vi "Read_tcx_file.vi"(8 "error in (no error)":errorcluster, 11 "file path":path) -> (0 "error out":errorcluster, 2 "Bpm":i32[](array[numeric]), 3 "Time":timestamp[](array[timestamp]))   [LabVIEW 2025]
uses:
  <vilib>/regexp/Match Regular Expression.xnode
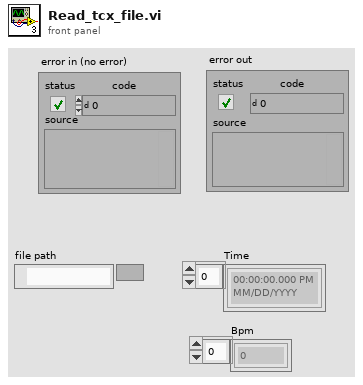
[diagram p1: front panel]
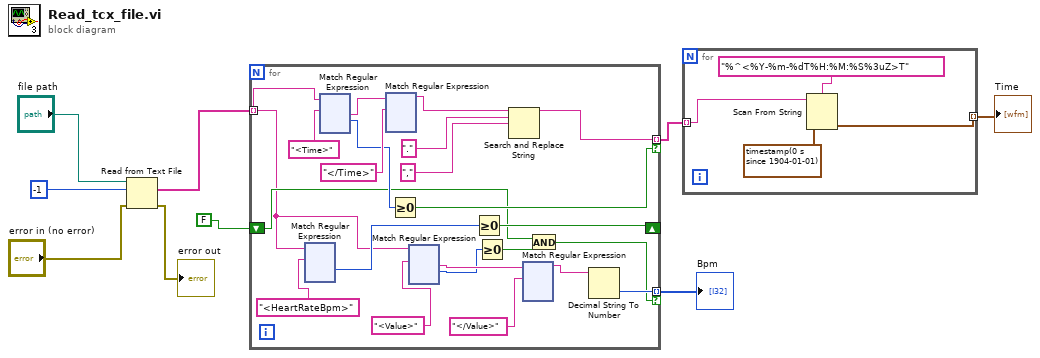
[diagram p0: block diagram]
diagram:
  n1 = Read from Text File(file (use dialog)="file path", count=-1, error in="error in (no error)") -> (text=w7:string[], error out=→"error out":errorcluster)  [unwired: 1 in, 2 out]
  n2 = for {
    tunnel: w7 -> [w10] mode=indexing
    tunnel: [w12] -> w2 mode=indexing if=w24
    shift-right: [w19] -> _
    shift-left: FALSE -> [w16]
    tunnel: [w14] -> w3 mode=indexing if=w13
    n3 = xnode "Match Regular Expression"("input string"=w10, "regular expression"="<HeartRateBpm>") -> ("offset past match"=w11:i32)  [unwired: 4 in, 4 out]
    n4 = xnode "Match Regular Expression"("input string"=w10, "regular expression"="<Time>") -> ("after match"=w30:string, "offset past match"=w25:i32)  [unwired: 4 in, 3 out]
    n5 = xnode "Match Regular Expression"("input string"=w30, "regular expression"="</Time>") -> ("before match"=w28:string)  [unwired: 4 in, 4 out]
    n6 = Greater Or Equal To 0?(x=w25) -> (x >= 0?=w24:bool)
    n7 = xnode "Match Regular Expression"("input string"=w10, "regular expression"="<Value>") -> ("after match"=w21:string, "offset past match"=w17:i32)  [unwired: 4 in, 3 out]
    n8 = Greater Or Equal To 0?(x=w11) -> (x >= 0?=w19:bool)
    n9 = Greater Or Equal To 0?(x=w17) -> (x >= 0?=w15:bool)
    n10 = Search and Replace String(input string=w28, search string=".", replace string=",") -> (result string=w12:string)  [unwired: 5 in, 3 out]
    n11 = xnode "Match Regular Expression"("input string"=w21, "regular expression"="</Value>") -> ("before match"=w18:string)  [unwired: 4 in, 4 out]
    n12 = And(x=w16, y=w15) -> (x .and. y?=w13:bool)
    n13 = Decimal String To Number(string=w18) -> (number=w14:i32)  [unwired: 2 in, 1 out]
  }
  "Bpm" <- w3
  n14 = for {
    tunnel: w2 -> [w619] mode=indexing
    tunnel: [w618] -> w1 mode=indexing
    n15 = Scan From String(format string="%^<%Y-%m-%dT%H:%M:%S%3uZ>T", input string=w619, default 1=timestamp(0 s since 1904-01-01)) -> (output 1=w618:timestamp)  [unwired: 2 in, 3 out]
  }
  "Time" <- w1
